vi "Get Device Parameters.vi"(8 "error in":errorcluster, 11 "Ballard ARINC 429 custom device in":T3=18446744073709551615 format="%.0x") -> (0 "error out":errorcluster, 2 "device parameters":T1, 3 "Ballard ARINC 429 custom device out":T3 format="%.0x")   [LabVIEW 2020, in "Ballard ARINC 429 Scripting.lvlib"]
doc: "Returns Ballard hardware device parameters such as <b>PXI slot number</b> and <b>core number</b>."
uses:
  Ballard ARINC 429 Scripting.lvlib
  <vilib>/NI VeriStand/Custom Device API/Custom Device Item Ref.ctl
  Shared/Device Parameters.ctl
  Shared/Initialization Method.ctl
  Constants.vi
  <vilib>/NI VeriStand/Custom Device API/Get Item Property (I32).vi
  <vilib>/NI VeriStand/Custom Device API/Get Item Property (U16).vi
  <vilib>/NI VeriStand/Custom Device API/Custom Device API.lvlib
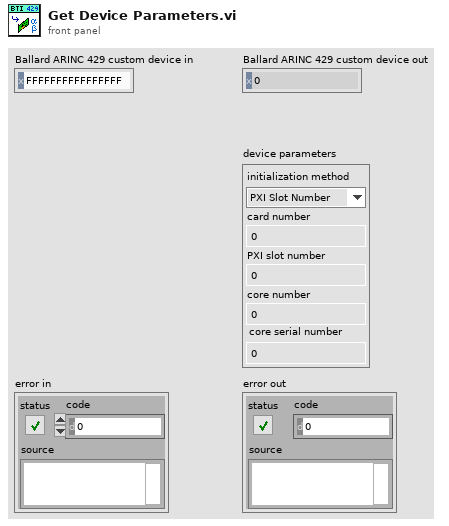
[diagram p1: front panel]
types:
  T1 = typedef "Device Parameters.ctl" = cluster{"initialization method":T2, "card number":i32, "PXI slot number":i32, "core number":i32, "core serial number":i32}
  T2 = typedef "Initialization Method.ctl" = enum16{"PXI Slot Number", "Card Number", "Core Serial Number"}
  T3 = typedef "Custom Device API.lvlib/Custom Device Item Ref.ctl" = u64
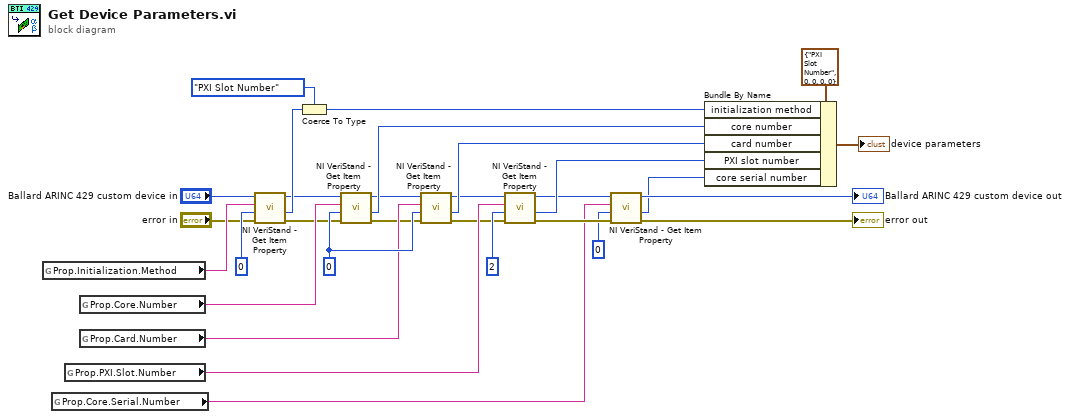
[diagram p0: block diagram]
diagram:
  w28 = 0 ("Default Value")
  n1 = global read "Constants.vi" "Prop.Initialization.Method"() -> (w23:string)
  n2 = global read "Constants.vi" "Prop.Core.Serial.Number"() -> (w3:string)
  n3 = global read "Constants.vi" "Prop.PXI.Slot.Number"() -> (w24:string)
  n4 = global read "Constants.vi" "Prop.Core.Number"() -> (w26:string)
  n5 = global read "Constants.vi" "Prop.Card.Number"() -> (w25:string)
  n6 = call-poly <vilib>:"NI VeriStand - Get Item Property.vi"("error in (no error)"="error in", "Default Value"=u16 0, "Property Name"=w23, "Item Ref in"="Ballard ARINC 429 custom device in") -> ("error out"=w10:errorcluster, "Value"=w19:u16, "Item Ref out"=w9:T3)  [unwired: 4 in, 1 out]
  n7 = Coerce To Type(0:w19, 1:Initialization_Method."PXI Slot Number" ("initialization method")) -> (2:w8:T2)
  n8 = call-poly <vilib>:"NI VeriStand - Get Item Property.vi"("error in (no error)"=w10, "Default Value"=w28, "Property Name"=w26, "Item Ref in"=w9) -> ("error out"=w16:errorcluster, "Value"=w22:i32, "Item Ref out"=w17:T3)  [unwired: 4 in, 1 out]
  n9 = call-poly <vilib>:"NI VeriStand - Get Item Property.vi"("error in (no error)"=w16, "Default Value"=w28, "Property Name"=w25, "Item Ref in"=w17) -> ("error out"=w14:errorcluster, "Value"=w21:i32, "Item Ref out"=w15:T3)  [unwired: 4 in, 1 out]
  n10 = call-poly <vilib>:"NI VeriStand - Get Item Property.vi"("error in (no error)"=w14, "Default Value"=2, "Property Name"=w24, "Item Ref in"=w15) -> ("error out"=w7:errorcluster, "Value"=w20:i32, "Item Ref out"=w5:T3)  [unwired: 4 in, 1 out]
  n11 = call-poly <vilib>:"NI VeriStand - Get Item Property.vi"("error in (no error)"=w7, "Default Value"=0, "Property Name"=w3, "Item Ref in"=w5) -> ("error out"=→"error out":errorcluster, "Value"=w1:i32, "Item Ref out"=→"Ballard ARINC 429 custom device out":T3)  [unwired: 4 in, 1 out]
  n12 = Bundle By Name(cluster=T1 {"initialization method"=enum."PXI Slot Number", "card number"=0, "PXI slot number"=0, "core number"=0, "core serial number"=0} ("device parameters"), "initialization method"=w8, "core number"=w22, "card number"=w21, "PXI slot number"=w20, "core serial number"=w1) -> (→"device parameters":T1)
